vi "Target.vi"() -> ()   [LabVIEW 2018]
uses:
  <vilib>/Platform/TimedLoop/XDataNode/timing_clust.ctl
  <vilib>/Platform/TimedLoop/XDataNode/nitl_modes.ctl
  <vilib>/Platform/TimedLoop/XDataNode/wakeup.ctl
  <vilib>/rvi/eio/common/nirviEmuTemplateMethod_errors.vi
  <vilib>/rvi/Emulation/niFpgaSctlEmulationGetInTimedLoop.vi
  <vilib>/rvi/Emulation/niFpgaEmulationReportErrorSimple.vi
  <vilib>/rvi/Emulation/niFpgaGetClockAttributes.vi
  <vilib>/rvi/Emulation/niFpgaCriticalErrorInLSC.vi
  <vilib>/rvi/Emulation/niFpgaProcessEmulError.vi
  <vilib>/eio/EIONode/EIONode.xnode
  <vilib>/Platform/TimedLoop/XDataNode/XDataNode.xnode
  <vilib>/Platform/TimedLoop/XDataNode/XDNodeRunTimeDep.lvlib
panel:
  in  "CR":bool[](array[boolean])=[TRUE, TRUE, TRUE, TRUE, FALSE, TRUE, TRUE, FALSE]
  in  "641":u16=641
  in  "17":u16=17
  in  "RS (CR=T)":bool
  in  "SEL":bool=TRUE
  out "DOUT":bool
  in  "DR":bool[](array[boolean])=[TRUE, FALSE, FALSE, TRUE, FALSE, TRUE, FALSE, FALSE, FALSE, FALSE, TRUE, TRUE, FALSE, FALSE, FALSE, FALSE, FALSE, FALSE, FALSE, FALSE, FALSE, FALSE, FALSE, FALSE, TRUE, FALSE, FALSE, FALSE, FALSE, FALSE, FALSE, FALSE, TRUE, FALSE, FALSE, FALSE, FALSE, FALSE, FALSE, TRUE, FALSE, FALSE, FALSE, FALSE, FALSE, FALSE, FALSE, FALSE, FALSE, FALSE, FALSE, FALSE, FALSE, FALSE, FALSE, FALSE, FALSE, FALSE, FALSE, FALSE, FALSE, FALSE, FALSE, FALSE, FALSE, FALSE, FALSE, FALSE, FALSE, FALSE, FALSE, FALSE, FALSE, FALSE, FALSE, FALSE, FALSE, FALSE, FALSE, FALSE, FALSE, FALSE, FALSE, FALSE, FALSE, FALSE, FALSE, FALSE, FALSE, FALSE, FALSE, FALSE, FALSE, FALSE, FALSE, FALSE, FALSE, FALSE, FALSE, FALSE, FALSE, FALSE, FALSE, FALSE, FALSE, FALSE, FALSE, FALSE, FALSE, FALSE, FALSE, FALSE, FALSE, FALSE, FALSE, FALSE, FALSE, FALSE, FALSE, FALSE, FALSE, FALSE, FALSE, FALSE, FALSE, FALSE, FALSE, FALSE, FALSE, FALSE, FALSE, FALSE, FALSE, FALSE, FALSE, FALSE, FALSE, FALSE, FALSE, FALSE, FALSE, FALSE, FALSE, FALSE, FALSE, FALSE, FALSE, FALSE, FALSE, FALSE, FALSE, FALSE, FALSE, FALSE, FALSE, FALSE, FALSE, FALSE, FALSE, FALSE, FALSE, FALSE, FALSE, FALSE, FALSE, FALSE, FALSE, FALSE, FALSE, FALSE, FALSE, FALSE, FALSE, FALSE, FALSE, FALSE, FALSE, FALSE, FALSE, FALSE, FALSE, FALSE, FALSE, FALSE, FALSE, FALSE, FALSE, FALSE, FALSE, FALSE, FALSE, FALSE, FALSE, FALSE, FALSE, FALSE, FALSE, FALSE, FALSE, FALSE, FALSE, FALSE, FALSE, FALSE, FALSE, FALSE, FALSE, FALSE, FALSE, FALSE, FALSE, FALSE, FALSE, FALSE, FALSE, FALSE, FALSE, FALSE, FALSE, FALSE, FALSE, FALSE, FALSE, FALSE, FALSE, FALSE, FALSE, FALSE, FALSE, FALSE, FALSE, FALSE, FALSE, FALSE, FALSE, FALSE, FALSE, FALSE, FALSE, FALSE, FALSE, FALSE, FALSE, FALSE, FALSE, FALSE, FALSE, FALSE, FALSE, FALSE, FALSE, FALSE, FALSE, FALSE, FALSE, FALSE, FALSE, FALSE, FALSE, FALSE, FALSE, FALSE, FALSE, FALSE, FALSE, FALSE, FALSE, FALSE, FALSE, FALSE, FALSE, FALSE, FALSE, FALSE, FALSE, FALSE, FALSE, FALSE, FALSE, FALSE, FALSE, FALSE, FALSE, FALSE, FALSE, FALSE, FALSE, FALSE, FALSE, FALSE, FALSE, FALSE, FALSE, FALSE, FALSE, FALSE, FALSE, FALSE, FALSE, FALSE, FALSE, FALSE, FALSE, FALSE, FALSE, FALSE, FALSE, FALSE, FALSE, FALSE, FALSE, FALSE, FALSE, FALSE, FALSE, FALSE, FALSE, FALSE, FALSE, TRUE]
  in  "Запись":bool
  in  "nRESET":bool=TRUE
  in  "BLANK":bool
  in  "Stop_FPGA":bool
  # "0"
  # "7"
  # "H"
  # "H"
  # "H"
  # "H"
  # "H"
  # "H"
  # "High - normal operation"
  # "Set Low to select Word 0"
  # "Яркость"
  # "Ток"
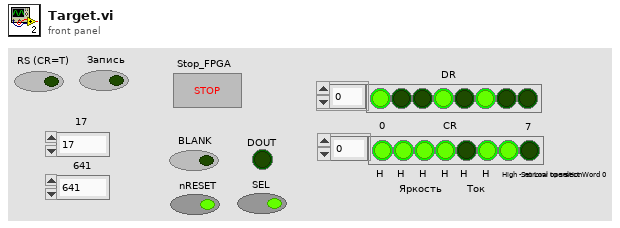
[diagram p1: front panel]
types:
  T1 = typedef "XDNodeRunTimeDep.lvlib/timing_clust.ctl" = cluster{"Expected End [f-1]":u64, "Actual End [f-1]":u64, "Finished Late? [f-1]":bool, "Expected End [i-1]":u64, "Actual End [i-1]":u64, "Finished Late? [i-1]":bool, "Expected Start [i]":u64, "Actual Start [i]":u64, "Expected Start [f]":u64, "Actual Start [f]":u64, "Source Name":string, "Structure Name":string, "Period":i64, "Deadline":i64, "Offset":i64, "Start":i64, "Priority":i32, "Timeout":i32, "Mode":T2, "Wakeup Reason":T3, "Error":errorcluster, "Source Type":string, "Secondary Source Type":string, "Global End Time":u64, "Global Start Time":u64, "Frame Duration":u64, "Iteration Duration":u64, "Assigned CPU":i32, "I/O Scan Engine Mode":u32}
  T2 = typedef "XDNodeRunTimeDep.lvlib/nitl_modes.ctl" = enum32{"No Change", "Process missed periods, maintain original phase", "Discard missed periods, maintain original phase", "Process missed periods, ignore original phase", "Discard missed periods, ignore original phase"}
  T3 = typedef "XDNodeRunTimeDep.lvlib/wakeup.ctl" = enum32{"Normal", "Aborted", "Asynchronous wakeup", "Timing source error", "Timed loop error", "Timeout"}
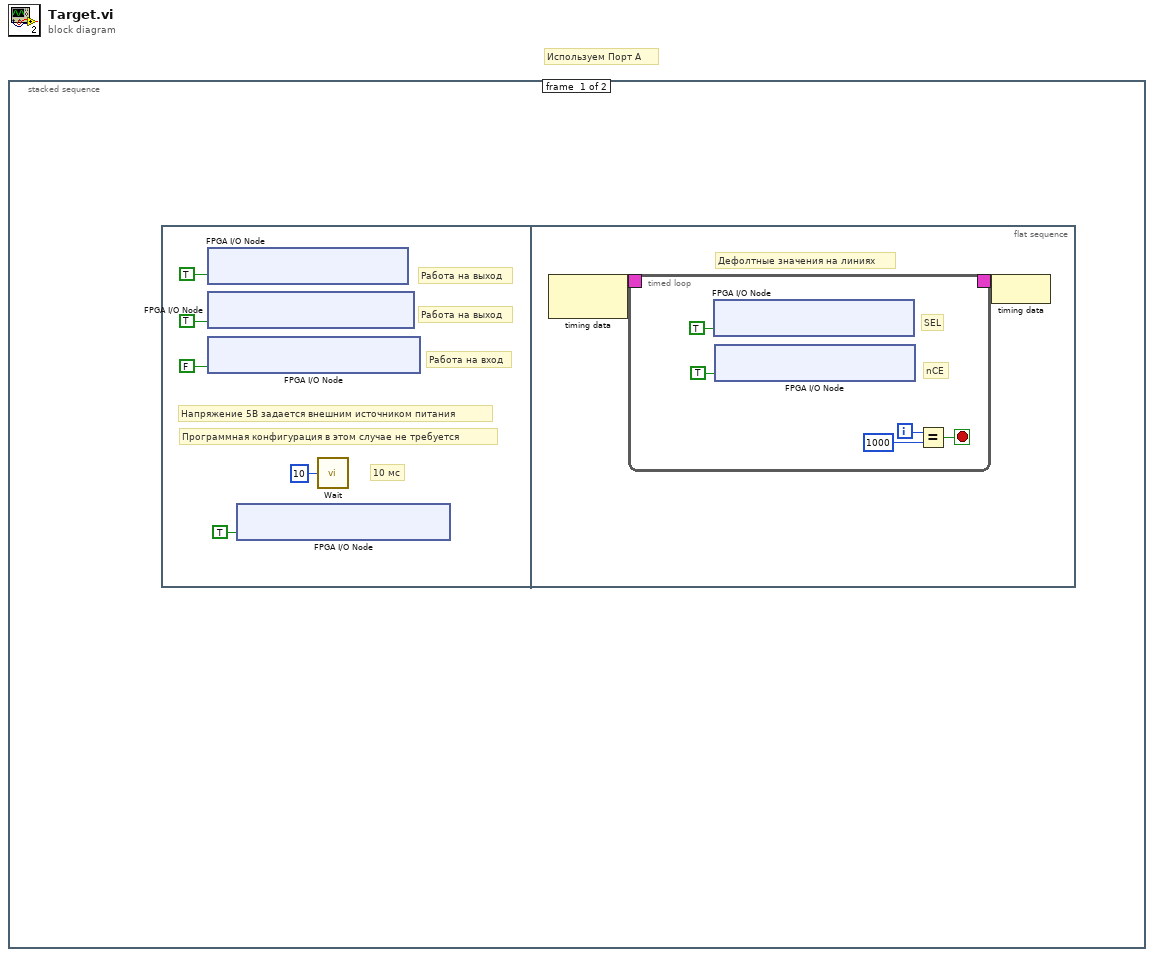
[diagram p0: block diagram]
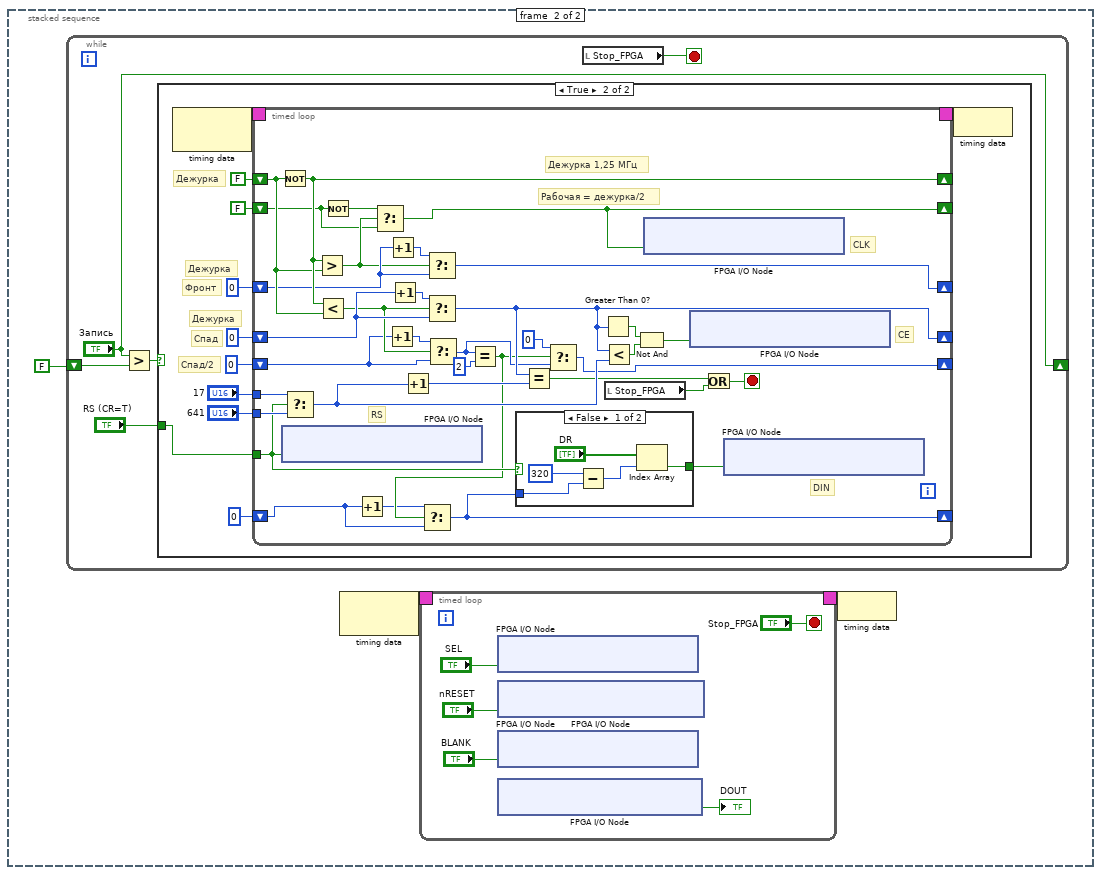
[diagram p2: hidden frame]
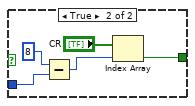
[diagram p4: hidden frame]
diagram:
  # "Используем Порт А"
  n1 = stacked-sequence {
    frame #0 {
      n2 = flat-sequence {
        frame #0 {
          # "Работа на вход"
          # "Программная конфигурация в этом случае не требуется"
          # "Напряжение 5В задается внешним источником питания"
          # "Работа на выход"
          # "10 мс"
          # "Работа на выход"
          n3 = xnode "FPGA I/O Node"("IO Module\\DDCA_DIO0-7_WE"=TRUE ("IO Module\\DDCA_DIO0-7_WE")) -> ()  [unwired: 1 in, 1 out]
          n4 = xnode "FPGA I/O Node"("IO Module\\DDCA_DIO8-15_WE"=TRUE ("IO Module\\DDCA_DIO8-15_WE")) -> ()  [unwired: 1 in, 1 out]
          n5 = xnode "FPGA I/O Node"("IO Module\\DDCA_DIO16-23_WE"=FALSE ("IO Module\\DDCA_DIO8-15_WE")) -> ()  [unwired: 1 in, 1 out]
          n6 = xnode "FPGA I/O Node"("IO Module\\DDCA_Supply_Select"=TRUE ("IO Module\\DDCA_Supply_Select")) -> ()  [unwired: 1 in, 1 out]
          n7 = call "Wait"("Count(mSec)"=u8 10 ("Count(uSec)")) -> ()  [unwired: 1 out]
        }
        frame #1 {
          # "Дефолтные значения на линиях"
          n8 = node-c288() -> (w7:T1)  [unwired: 1 in]
          n9 = timed-loop {
            timing: w7 -> [_]
            timing-out: [_] -> w6
            i -> [w11]
            stop <- w12 stop-if-true
            # "SEL"
            # "nCE"
            n10 = xnode "FPGA I/O Node"("IO Module\\DDCA_DIO8_Write"=TRUE ("IO Module\\DDCA_DIO8_Write")) -> ()  [unwired: 1 in, 1 out]
            n11 = xnode "FPGA I/O Node"("IO Module\\DDCA_DIO4_Write"=TRUE ("IO Module\\DDCA_DIO4_Write")) -> ()  [unwired: 1 in, 1 out]
            n12 = Equal?(x=w11, y=1000) -> (x = y?=w12:bool)
          }
          n13 = node-c288(w6) -> ()
        }
      }
    }
    frame #1 {
      n14 = while {
        shift-right: ["Запись"] -> _
        shift-left: FALSE ("SPI") -> [w32]
        stop <- w30 stop-if-true
        n15 = Greater?(x="Запись", y=w32) -> (0:w33:bool)
        n16 = case shown="True" w33 {
          tunnel: "RS (CR=T)" -> [_ w42]
          frame False {
          }
          frame True {
            # "Спад/2"
            # "Дежурка"
            # "Дежурка"
            # "Дежурка"
            # "Спад"
            # "Фронт"
            n17 = node-c288() -> (w44:T1)  [unwired: 1 in]
            n18 = timed-loop {
              timing: w44 -> [_]
              timing-out: [_] -> w43
              tunnel: w42 -> [w63]
              shift-right: [w79] -> _
              shift-left: FALSE -> [w78]
              shift-right: [w61] -> _
              shift-left: u16 0 -> [w73]
              shift-right: [w75] -> _
              shift-left: u16 0 -> [w77]
              tunnel: "17" -> [w72]
              tunnel: "641" -> [w71]
              shift-right: [w67] -> _
              shift-left: FALSE -> [w68]
              shift-right: [w49] -> _
              shift-left: u8 0 -> [w53]
              shift-right: [w45] -> _
              shift-left: u16 0 -> [w46]
              stop <- w57 stop-if-true
              # "Рабочая = дежурка/2"
              # "Дежурка 1,25 МГц"
              # "CE"
              # "CLK"
              # "RS"
              # "DIN"
              n19 = Not(x=w78) -> (.not. x?=w79:bool)
              n20 = xnode "FPGA I/O Node"("IO Module\\DDCA_DIO1_Write"=w63) -> ()  [unwired: 1 in, 1 out]
              n21 = Select(t=w72, s=w63, f=w71) -> (s? t:f=w60:u16)
              n22 = Greater?(x=w79, y=w78) -> (0:w70:bool)
              n23 = Less?(x=w79, y=w78) -> (x < y?=w55:bool)
              n24 = Not(x=w68) -> (.not. x?=w69:bool)
              n25 = Increment(x=w46) -> (x+1=w47:u16)
              n26 = Select(t=w69, s=w70, f=w68) -> (s? t:f=w67:bool)
              n27 = Increment(x=w53) -> (x+1=w54:u8)
              n28 = Increment(x=w77) -> (x+1=w76:u16)
              n29 = Increment(x=w73) -> (x+1=w74:u16)
              n30 = Increment(x=w60) -> (x+1=w56:u16)
              n31 = Select(t=w76, s=w70, f=w77) -> (s? t:f=w75:u16)
              n32 = Select(t=w74, s=w55, f=w73) -> (s? t:f=w61:u16)
              n33 = Select(t=w54, s=w55, f=w53) -> (s? t:f=w50:u8)
              n34 = Equal?(x=w50, y=u8 2) -> (x = y?=w48:bool)
              n35 = Select(t=w47, s=w48, f=w46) -> (s? t:f=w45:u16)
              n36 = case shown="False" w63 {
                tunnel: w45 -> [w80 w86]
                tunnel: [w84 w88] -> w62
                frame False {
                  n37 = Subtract(x=u16 320, y=w80) -> (x-y=w82:u16)
                  n38 = Index Array(array="DR", index=w82) -> (element=w84:bool)
                }
                frame True {
                  n39 = Subtract(x=u16 8, y=w86) -> (x-y=w85:u16)
                  n40 = Index Array(array="CR", index=w85) -> (element=w88:bool)
                }
              }
              n41 = Equal?(x=w61, y=w56) -> (x = y?=w59:bool)
              n42 = Select(t=u8 0, s=w48, f=w50) -> (s? t:f=w49:u8)
              n43 = Greater Than 0?(x=w61) -> (x > 0?=w66:bool)
              n44 = Less?(x=w61, y=w60) -> (x < y?=w65:bool)
              n45 = local read "Stop_FPGA"() -> (w58:bool)
              n46 = Not And(1:w65, 2:w66) -> (0:w64:bool)
              n47 = xnode "FPGA I/O Node"("IO Module\\DDCA_DIO3_Write"=w67) -> ()  [unwired: 1 in, 1 out]
              n48 = xnode "FPGA I/O Node"("IO Module\\DDCA_DIO4_Write"=w64) -> ()  [unwired: 1 in, 1 out]
              n49 = Or(x=w59, y=w58) -> (x .or. y?=w57:bool)
              n50 = xnode "FPGA I/O Node"("IO Module\\DDCA_DIO0_Write"=w62) -> ()  [unwired: 1 in, 1 out]
            }
            n51 = node-c288(w43) -> ()
          }
        }
        n52 = local read "Stop_FPGA"() -> (w30:bool)
      }
      n53 = node-c288() -> (w19:T1)  [unwired: 1 in]
      n54 = timed-loop {
        timing: w19 -> [_]
        timing-out: [_] -> w18
        stop <- "Stop_FPGA" stop-if-true
        n55 = xnode "FPGA I/O Node"("IO Module\\DDCA_DIO8_Write"="SEL") -> ()  [unwired: 1 in, 1 out]
        n56 = xnode "FPGA I/O Node"("IO Module\\DDCA_DIO14_Write"="nRESET") -> ()  [unwired: 1 in, 1 out]
        n57 = xnode "FPGA I/O Node"("IO Module\\DDCA_DIO6_Write"="BLANK") -> ()  [unwired: 1 in, 1 out]
        n58 = xnode "FPGA I/O Node"() -> ("IO Module\\DDCA_DIO16_Read"=→"DOUT":bool)  [unwired: 1 in, 1 out]
      }
      n59 = node-c288(w18) -> ()
    }
  }
